vi "Get SMO Serial Number.vi"(8 "error in (no error)":errorcluster, 11 "Instrument.Lockin in":refnum<class "Instrument.Lockin.lvclass">) -> (0 "error out":errorcluster, 2 "Serial Number":string, 3 "Instrument.Lockin out":refnum<class "Instrument.Lockin.lvclass">)   [LabVIEW 2019, in "Instrument.Lockin.lvlib" / "Instrument.Lockin.lvclass"]
doc: "Override this VI to return the serial number of your Instrument"
uses:
  Instrument.Lockin.lvclass
  Instrument.Lockin.lvclass/Instrument.Lockin.ctl
  fe1946f7-5328-434b-bdcb-a523eae19b2f.vi
  <userlib>/LevyLab/Instrument Framework/Instrument Types/Lockin/Instrument.LockinAPI.lvclass
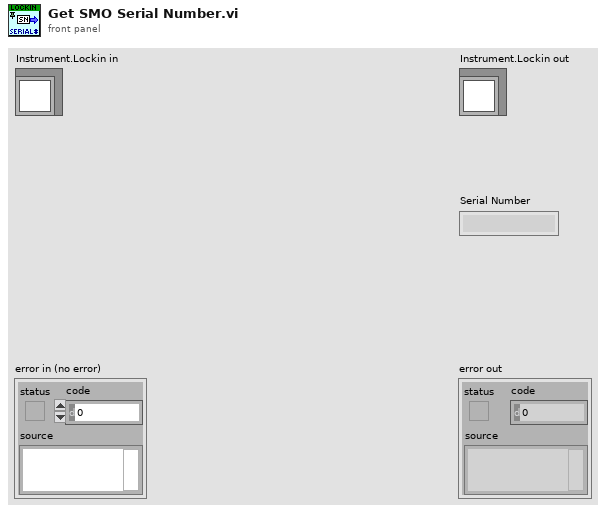
[diagram p1: front panel]
types:
  T1 = typedef "Instrument.Lockin.lvlib/Instrument.DAQ.lvclass/DeviceInfo--Cluster.ctl" = cluster{"DeviceName":string, "DevIsSimulated":bool, "DeviceSerialNumber":string, "ProductType":string, "ProductCategory":i32, "ProductNumber":u32, "ChassisNumber":u32, "SlotNumber":u32, "ChassisName":string, "ChassisSerialNumber":string, "DevTemp":dbl, "SelfCal.LastDate/Time":string, "SelfCal.LastTemp":dbl, "calibration due?":bool}
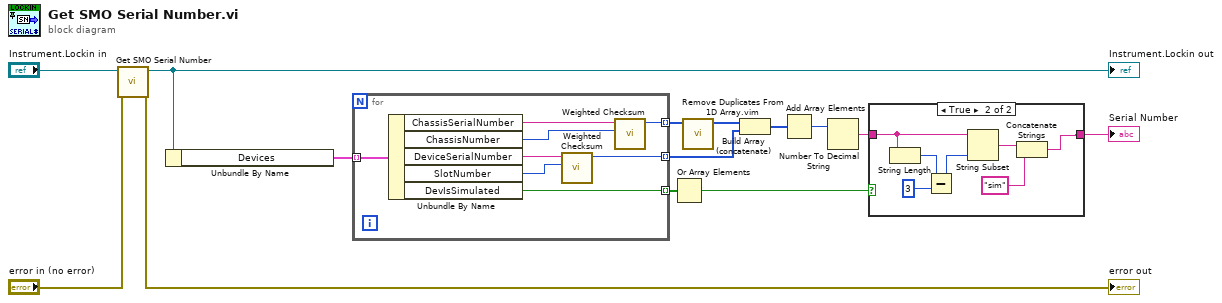
[diagram p0: block diagram]
diagram:
  n1 = call-parent "Get SMO Serial Number.vi"("error in (no error)"="error in (no error)", "Instrument in"="Instrument.Lockin in") -> ("error out"=→"error out":errorcluster, "Instrument out"=w13:refnum<class "Instrument.Lockin.lvclass">)  [unwired: 7 in, 1 out]
  "Instrument.Lockin out" <- w13
  n2 = Unbundle By Name(w13) -> ("Devices"=w10:T1[])
  n3 = for {
    tunnel: w10 -> [w22] mode=indexing
    tunnel: [w17] -> w9 mode=indexing
    tunnel: [w16] -> w7 mode=indexing
    tunnel: [w15] -> w2 mode=indexing
    n4 = Unbundle By Name(w22) -> ("ChassisSerialNumber"=w19:string, "ChassisNumber"=w18:u32, "DeviceSerialNumber"=w21:string, "SlotNumber"=w20:u32, "DevIsSimulated"=w15:bool)
    n5 = call "Weighted Checksum.vi"("Weight"=w20, "Text"=w21) -> ("Checksum"=w16:u32)  [unwired: 9 in]
    n6 = call "Weighted Checksum.vi"("Weight"=w18, "Text"=w19) -> ("Checksum"=w17:u32)  [unwired: 9 in]
  }
  n7 = Or Array Elements(Boolean array=w2) -> (logical OR=w1:bool)
  n8 = call "Remove Duplicates From 1D Array.vim"("array"=w9) -> ("array with duplicates removed"=w8:u32[])  [unwired: 10 in]
  n9 = Build Array (concatenate)(w8, w7) -> (w6:u32[])
  n10 = Add Array Elements(numeric array=w6) -> (sum=w5:u32)
  n11 = Number To Decimal String(number=w5) -> (decimal integer string=w4:string)  [unwired: 1 in]
  n12 = case shown="True" w1 {
    tunnel: w4 -> [w23 w25]
    tunnel: [w23 w24] -> w3
    frame False {
    }
    frame True {
      n13 = String Length(string=w25) -> (length=w30:i32)
      n14 = Subtract(x=w30, y=3) -> (x-y=w28:i32)
      n15 = String Subset(string=w25, length (rest)=w28) -> (substring=w27:string)  [unwired: 1 in]
      n16 = Concatenate Strings(w27, "sim" ("string")) -> (w24:string)
    }
  }
  "Serial Number" <- w3
